vi "Initialization.vi"(8 "error in":errorcluster, 9 "UI Refs":T1, 10 "user event":T2, 11 "H1 Velocity":refnum<class "H1 Velocity.lvclass">) -> (0 "error out":errorcluster, 3 "H1 Velocity out":refnum<class "H1 Velocity.lvclass">)   [LabVIEW 2025, in "H1 Plotter.lvlib" / "H1 Velocity.lvclass"]
uses:
  H1 Velocity.lvclass
  Users/Public/Documents/Sandia National Labs/TSS Plugin/CEF.lvlibp/Node/UserEventRef.ctl
  Users/Public/Documents/Sandia National Labs/TSS Plugin/Tests/XY Plotter.lvlibp/XY  Plotter/XY Plotter.lvclass
  H1 Velocity.lvclass/H1 Velocity.ctl
  Users/Public/Documents/Sandia National Labs/TSS Plugin/CEF.lvlibp/Node/CEF_Node.lvclass
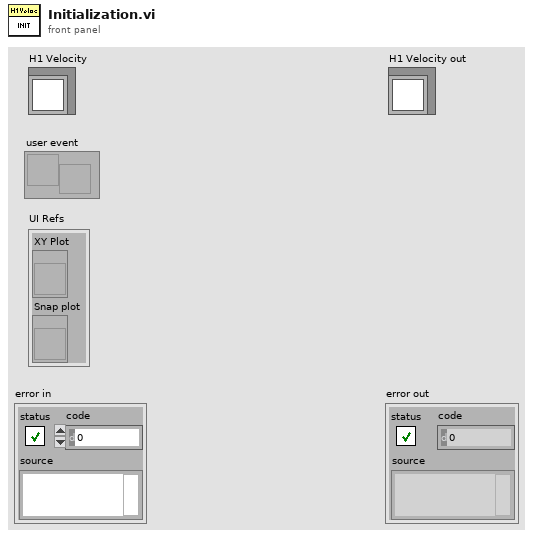
[diagram p1: front panel]
types:
  T1 = cluster{"XY Plot":refnum<vi>, "Snap plot":refnum<vi>}
  T2 = typedef "CEF.lvlibp/CEF_Node.lvclass/UserEventRef.ctl" = refnum<user-event>
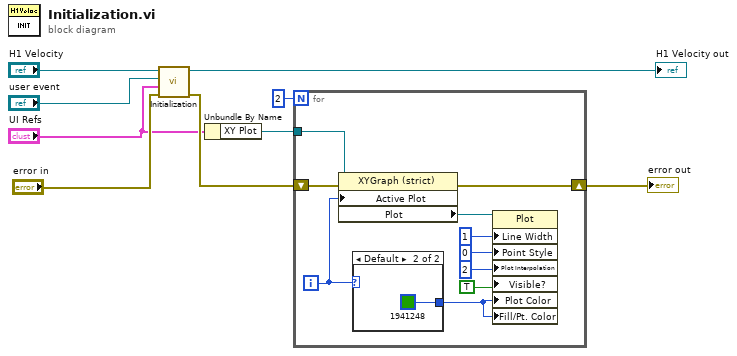
[diagram p0: block diagram]
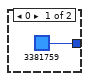
[diagram p2: hidden frame]
diagram:
  n1 = call-parent "Initialization.vi"("error in"="error in", "UI Refs"="UI Refs", "user event"="user event", "XY Plotter"="H1 Velocity") -> ("error out"=w5:errorcluster, "XY Plotter out"=→"H1 Velocity out":refnum<class "H1 Velocity.lvclass">)  [unwired: 6 in]
  n2 = Unbundle By Name("UI Refs") -> ("XY Plot"=w2:refnum<vi>)
  n3 = for {
    N: 2 -> [_]
    tunnel: w2 -> [w19]
    shift-right: [w10] -> w4
    shift-left: w5 -> [w14]
    i -> [w12]
    n4 = property class="XYGraph (strict)"(reference=w19, error in=w14, "Active Plot"=w12) -> (error out=w10:errorcluster, "Plot"=w15:refnum<vi>)  [unwired: 1 out]
    n5 = case shown="Default" w12 {
      tunnel: [u32 3381759 ("Plot Color") u32 1941248 ("Plot Color")] -> w11
      frame 0 {
      }
      frame Default {
      }
    }
    n6 = property class="Plot"(reference=w15, "Line Width"=u8 1, "Point Style"=u8 0, "Plot Interpolation"=u8 2, "Visible?"=TRUE ("Visible"), "Plot Color"=w11, "Fill/Pt. Color"=w11) -> ()  [unwired: 1 in, 2 out]
  }
  "error out" <- w4
